vi "RemoteVI Serve Clients Step.vi"(0 "state":T1, 5 "clients":T2(array[cluster]), 7 "track":T4, 9 "context":T3, 11 "error":errorcluster) -> (4 "state out":T1, 6 "clients out":T2(array[cluster]), 8 "captured?":bool, 10 "stopped?":bool)   [LabVIEW 2020, in "RemoteVI.lvlib"]
doc: "One iteration of the server loop, second half: serves the clients with what Track Target found. Service Clients reads and applies each client's input; Menu Hover follows a remote pointer over an open menu with keys; Retrack Popups lists the popups once more when a client posted something or a popup is open, so a popup the input just opened is hidden on the host at once and its overlay goes out before the frame; Click State keeps the displacement d and when a client last clicked. Then origin, tips and splitters go to the clients when they changed, the overlay (at once when the popups changed), a frame (Capture And Send, every 16 ms right after input), the other windows and the overlay again (150 ms period in a frame iteration). Closed clients are dropped, the status is published and VI Stopped checks once a second whether the shared VI still runs (only while VI Server may be called). stopped? is also TRUE as soon as the panel window that was shared no longer exists (user32 IsWindow.vi in every iteration, no VI Server call): a VI started over VI Server keeps running when its panel is closed, and the share would otherwise serve a window that is gone."
uses:
  RemoteVI.lvlib
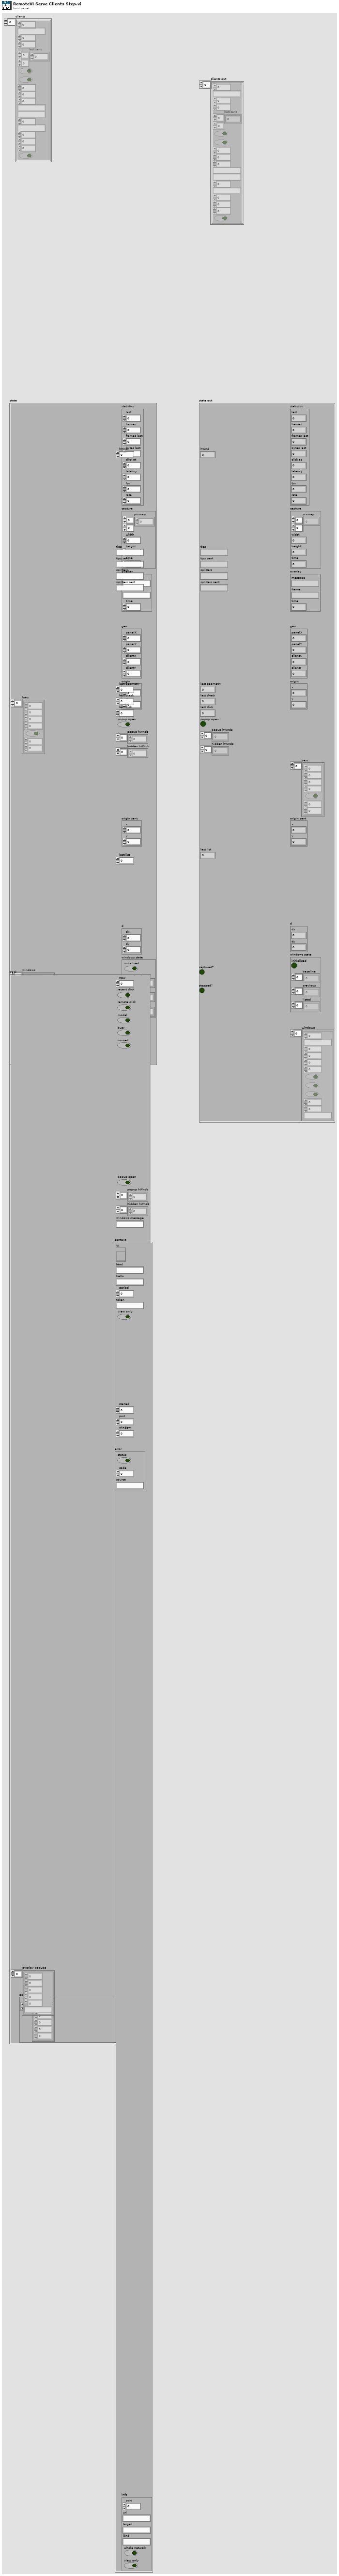
[diagram p1: front panel]
types:
  T1 = cluster{"statistics":cluster{"last":dbl, "frames":u32, "frames last":u32, "bytes last":dbl, "click at":dbl, "latency":dbl, "fps":dbl, "rate":dbl}, "capture":cluster{"pixmap":u32[][], "width":i32, "height":i32, "time":u32}, "overlay":cluster{"message":string, "frame":string, "time":u32}, "hWnd":u64, "geo":cluster{"panelX":i32, "panelY":i32, "clientX":i32, "clientY":i32}, "origin":cluster{"x":i32, "y":i32}, "tips":string, "tips sent":string, "splitters":string, "splitters sent":string, "bars":cluster{"x":i32, "y":i32, "w":i32, "h":i32, "vertical":bool, "min":i32, "max":i32}[], "origin sent":cluster{"x":i32, "y":i32}, "last geometry":u32, "last check":u32, "last click":u32, "popup open":bool, "popup hWnds":u64[], "hidden hWnds":u64[], "d":cluster{"dx":i32, "dy":i32}, "windows state":cluster{"initialised":bool, "baseline":u64[], "previous":u64[], "listed":u64[]}, "last list":u32, "windows":cluster{"id":u64, "title":string, "x":i32, "y":i32, "w":i32, "h":i32, "modal":bool, "active":bool, "closable":bool, "sx":i32, "sy":i32, "class":string}[]}
  T2 = cluster{"connection":u32, "rx buffer":string, "seq":u32, "acked":u32, "last sent":u32[][], "tracking":bool, "closed":bool, "mods":u8, "mods set":u8, "popup since":u32, "windows sent":string, "window frames":cluster{"id":u64, "pixels":u32[][]}[], "key window":u64, "address":string, "since":dbl, "last input":dbl, "bytes":dbl, "view only":bool}[]
  T3 = cluster{"VI":refnum<vi>, "html":string, "hello":string, "period":dbl, "token":string, "view only":bool, "info":cluster{"port":u16, "url":string, "target":string, "kind":string, "whole network":bool, "view only":bool}, "started":dbl, "port":u16, "window":u64}
  T4 = cluster{"now":u32, "recent click":bool, "remote click":bool, "modal":bool, "busy":bool, "moved":bool, "popups":cluster{"windows":cluster{"hwnd":u64, "x":i32, "y":i32, "w":i32, "h":i32}[], "dx":i32, "dy":i32}, "overlay popups":cluster{"hwnd":u64, "x":i32, "y":i32, "w":i32, "h":i32, "class":string}[], "popup open":bool, "popup hWnds":u64[], "hidden hWnds":u64[], "windows message":string}
  T5 = cluster{"windows":cluster{"hwnd":u64, "x":i32, "y":i32, "w":i32, "h":i32}[], "dx":i32, "dy":i32}
  T6 = cluster{"hwnd":u64, "x":i32, "y":i32, "w":i32, "h":i32, "class":string}[]
  T7 = cluster{"last":dbl, "frames":u32, "frames last":u32, "bytes last":dbl, "click at":dbl, "latency":dbl, "fps":dbl, "rate":dbl}
  T8 = cluster{"pixmap":u32[][], "width":i32, "height":i32, "time":u32}
  T9 = cluster{"message":string, "frame":string, "time":u32}
  T10 = cluster{"panelX":i32, "panelY":i32, "clientX":i32, "clientY":i32}
  T11 = cluster{"id":u64, "title":string, "x":i32, "y":i32, "w":i32, "h":i32, "modal":bool, "active":bool, "closable":bool, "sx":i32, "sy":i32, "class":string}[]
  T12 = cluster{"port":u16, "url":string, "target":string, "kind":string, "whole network":bool, "view only":bool}
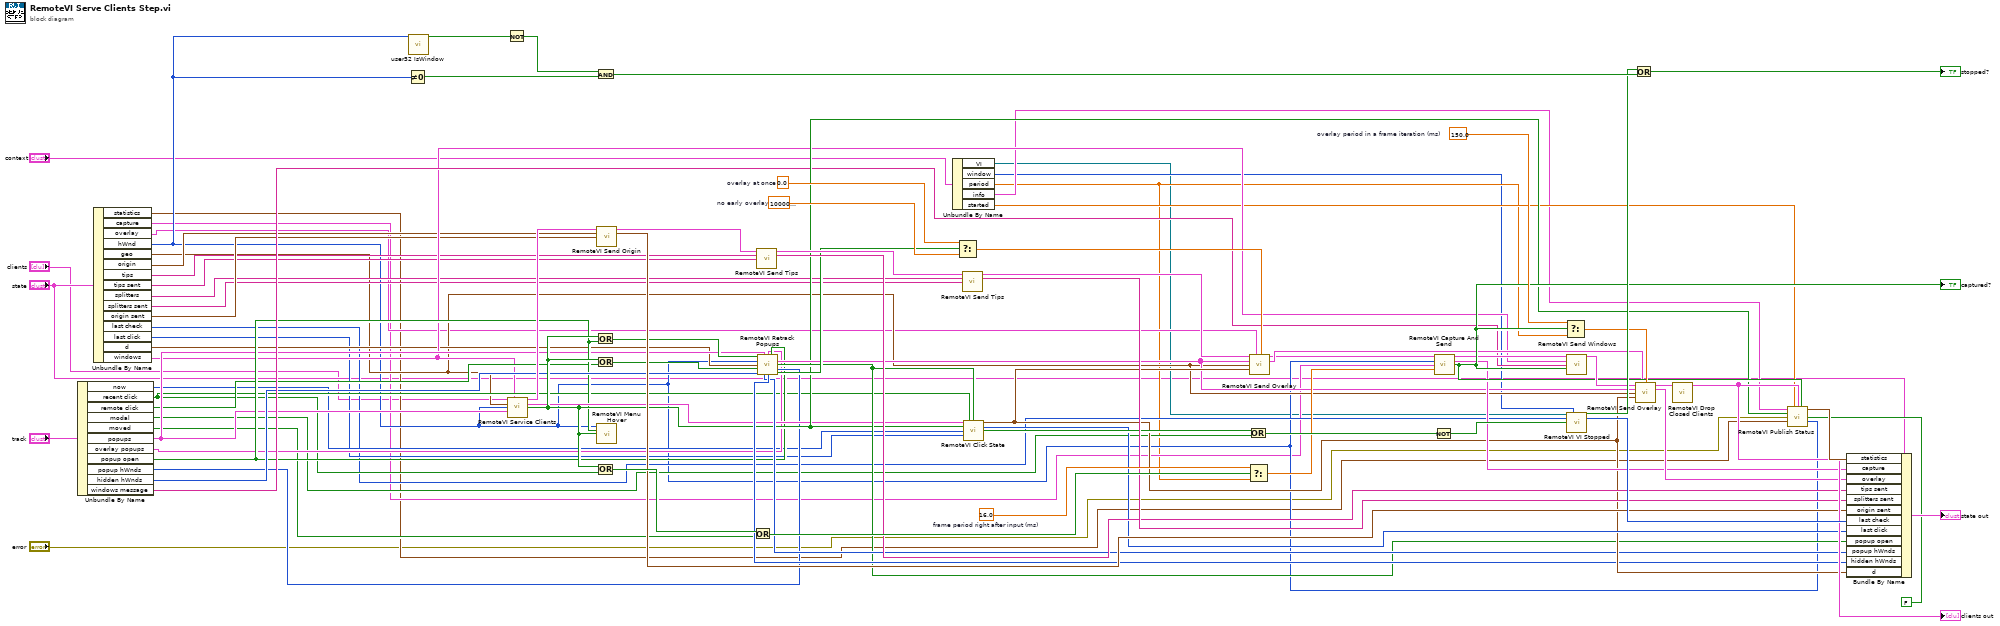
[diagram p0: block diagram]
diagram:
  w68 = 150.0  # overlay period in a frame iteration (ms)
  w61 = 16.0  # frame period right after input (ms)
  w57 = 1000000000.0  # no early overlay
  w56 = 0.0  # overlay at once
  n1 = Unbundle By Name("track") -> ("now"=w26:u32, "recent click"=w27:bool, "remote click"=w28:bool, "modal"=w29:bool, "moved"=w30:bool, "popups"=w31:T5, "overlay popups"=w32:T6, "popup open"=w33:bool, "popup hWnds"=w34:u64[], "hidden hWnds"=w35:u64[], "windows message"=w36:string)
  n2 = Unbundle By Name("state") -> ("statistics"=w11:T7, "capture"=w12:T8, "overlay"=w13:T9, "hWnd"=w14:u64, "geo"=w15:T10, "origin"=w16:cluster{"x":i32, "y":i32}, "tips"=w17:string, "tips sent"=w18:string, "splitters"=w19:string, "splitters sent"=w20:string, "origin sent"=w21:cluster{"x":i32, "y":i32}, "last check"=w22:u32, "last click"=w23:u32, "d"=w24:cluster{"dx":i32, "dy":i32}, "windows"=w25:T11)
  n3 = Not Equal To 0?(x=w14) -> (x != 0?=w83:bool)
  n4 = call "user32 IsWindow.vi"("hWnd"=w14) -> ("window?"=w81:bool)  [unwired: 13 in, 1 out]
  n5 = Not(x=w81) -> (.not. x?=w82:bool)
  n6 = call "RemoteVI Service Clients.vi"("clients"="clients", "windows"=w25, "geo"=w15, "hWnd"=w14, "popups"=w31) -> ("clients out"=w37:T2, "popups out"=w38:T5, "clicked?"=w39:bool)  [unwired: 8 in]
  n7 = Or(x=w39, y=w33) -> (x .or. y?=w40:bool)
  n8 = Or(x=w39, y=w28) -> (x .or. y?=w41:bool)
  n9 = Or(x=w39, y=w27) -> (x .or. y?=w62:bool)
  n10 = And(x=w82, y=w83) -> (x .and. y?=w84:bool)
  n11 = call "RemoteVI Send Origin.vi"("clients"=w37, "origin"=w16, "origin sent"=w21) -> ("clients out"=w50:T2, "origin sent out"=w51:cluster{"x":i32, "y":i32})  [unwired: 11 in]
  n12 = call "RemoteVI Menu Hover.vi"("hWnd"=w14, "popup open?"=w33, "clicked?"=w39) -> ()  [unwired: 13 in]
  n13 = Or(x=w62, y=w30) -> (x .or. y?=w63:bool)
  n14 = call "RemoteVI Send Tips.vi"("clients"=w50, "message"=w17, "message sent"=w18) -> ("clients out"=w52:T2, "message sent out"=w53:string)  [unwired: 11 in]
  n15 = call "RemoteVI Retrack Popups.vi"("again?"=w40, "popups"=w31, "overlay popups"=w32, "popup open?"=w33, "panel hWnd"=w14, "d"=w24, "remote click?"=w41, "popup hWnds"=w34, "hidden hWnds"=w35) -> ("overlay popups out"=w42:T6, "popup open? out"=w43:bool, "popup hWnds out"=w44:u64[], "hidden hWnds out"=w45:u64[], "changed?"=w46:bool)  [unwired: 1 in, 1 out]
  n16 = Unbundle By Name("context") -> ("VI"=w5:refnum<vi>, "window"=w6:u64, "period"=w7:dbl, "info"=w8:T12, "started"=w9:dbl)
  n17 = Select(t=w56, s=w46, f=w57) -> (s? t:f=w58:dbl)
  n18 = call "RemoteVI Send Tips.vi"("clients"=w52, "message"=w19, "message sent"=w20) -> ("clients out"=w54:T2, "message sent out"=w55:string)  [unwired: 11 in]
  n19 = call "RemoteVI Click State.vi"("popups out"=w38, "recent click?"=w27, "popup open?"=w43, "clicked?"=w39, "now"=w26, "last click"=w23) -> ("d"=w47:cluster{"dx":i32, "dy":i32}, "last click out"=w48:u32, "no VI Server?"=w49:bool)  [unwired: 7 in]
  n20 = Or(x=w49, y=w29) -> (x .or. y?=w76:bool)
  n21 = Select(t=w61, s=w63, f=w7) -> (s? t:f=w64:dbl)
  n22 = call "RemoteVI Send Overlay.vi"("clients"=w54, "state"=w13, "period"=w58, "overlay popups"=w42, "geo"=w15, "d"=w47) -> ("clients out"=w59:T2, "state out"=w60:T9)  [unwired: 8 in]
  n23 = Not(x=w76) -> (.not. x?=w77:bool)
  n24 = call "RemoteVI Capture And Send.vi"("clients"=w59, "hWnd"=w14, "cache"=w12, "period"=w64) -> ("clients out"=w65:T2, "cache out"=w66:T8, "captured?"=w67:bool)  [unwired: 9 in]
  "captured?" <- w67
  n25 = Select(t=w68, s=w67, f=w7) -> (s? t:f=w69:dbl)
  n26 = call "RemoteVI Send Windows.vi"("clients"=w65, "windows"=w25, "message"=w36, "capture?"=w67) -> ("clients out"=w70:T2)  [unwired: 11 in]
  n27 = call "RemoteVI VI Stopped.vi"("VI"=w5, "window"=w6, "last check"=w22, "VI Server ok?"=w77) -> ("stopped?"=w78:bool, "last check out"=w79:u32)  [unwired: 10 in]
  n28 = Or(x=w78, y=w84) -> (x .or. y?=→"stopped?":bool)
  n29 = call "RemoteVI Send Overlay.vi"("clients"=w70, "state"=w60, "period"=w69, "overlay popups"=w42, "geo"=w15, "d"=w47) -> ("clients out"=w71:T2, "state out"=w72:T9)  [unwired: 8 in]
  n30 = call "RemoteVI Drop Closed Clients.vi"("clients"=w71) -> ("clients out"=w73:T2)  [unwired: 14 in]
  "clients out" <- w73
  n31 = call "RemoteVI Publish Status.vi"("info"=w8, "started"=w9, "clients"=w73, "captured?"=w67, "clicked?"=w39, "error"="error", "stop?"=FALSE, "state"=w11, "hWnd"=w14) -> ("state out"=w75:T7)  [unwired: 6 in]
  n32 = Bundle By Name(cluster="state", "statistics"=w75, "capture"=w66, "overlay"=w72, "tips sent"=w53, "splitters sent"=w55, "origin sent"=w51, "last check"=w79, "last click"=w48, "popup open"=w43, "popup hWnds"=w44, "hidden hWnds"=w45, "d"=w47) -> (→"state out":T1)
